vi "UpdateClassApperance.vi"(0 "ClassRefIn":refnum<vi>, 2 "ClassType(Class)":T1, 5 "error in (no error)":errorcluster) -> (14 "ClassRefOut":refnum<vi>, 19 "error out":errorcluster)   [LabVIEW 2020, in "ClassWriter.lvclass"]
uses:
  ClassWriter.lvclass
  ClassApperanceType.ctl
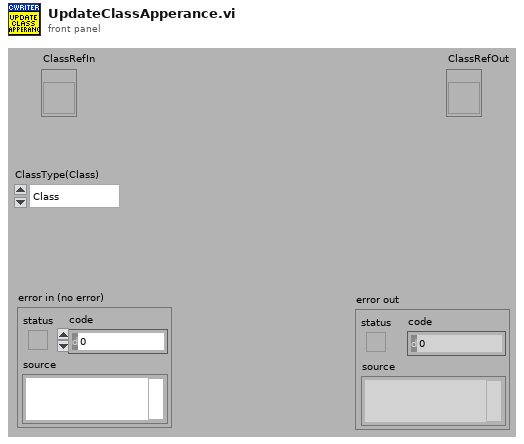
[diagram p1: front panel]
types:
  T1 = typedef "ClassApperanceType.ctl" = enum16{"Class", "AF-MessageClass", "Interface"}
  T2 = typedef "GOOP_WireConfigurationType.ctl" = cluster{"Edge thickness":i32, "Edge color":u32, "Center thickness":i32, "Center pattern":T3, "CenterColor1":u32, "CenterColor2":u32, "Tunnels and terminals colors":u32}
  T3 = typedef "GOOP_WirePattern.ctl" = enum16{"Solid", "Large dash", "Small dash"}
  T4 = typedef "BaseProvider_IniFileSettings.ctl" = cluster{"ClassFolderSuffix":string, "InterfaceFolderSuffix":string, "InterfaceIcon":string, "FileNamingOption":T5, "DynamicDispatchStartValue":bool}
  T5 = typedef "BaseProvider_FileNamingOption.ctl" = enum16{"CamelCase", "Space", "Underscore"}
  T6 = cluster{"Foreground Color":u32, "Background Color":u32, "Fill Pattern":cluster{"Row 0":u8, "Row 1":u8, "Row 2":u8, "Row 3":u8, "Row 4":u8, "Row 5":u8, "Row 6":u8, "Row 7":u8}, "Width":i16, "Mode":enum16{"Copy", "Or", "Exclusive Or", "Bit Clear", "Not Copy", "Not Or", "Nor Exclusive Or", "Not Bit Clear"}, "Style":enum32{"Solid", "Dash", "Dot", "Dash Dot", "Dash Dot Dot"}, "Fill Rule":enum32{"Even Odd", "Winding"}, "End Caps":enum32{"Default", "Flat"}}[]
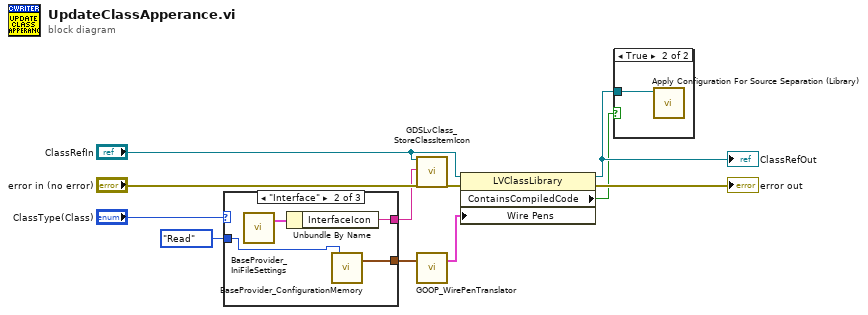
[diagram p0: block diagram]
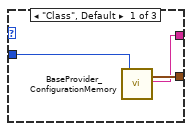
[diagram p3: hidden frame]
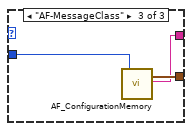
[diagram p4: hidden frame]
diagram:
  n1 = case shown="\"Interface\"" "ClassType(Class)" {
    tunnel: [w14 w18 w20] -> w11
    tunnel: [w13 w15 w19] -> w7
    tunnel: enum16{"Read", "Load", "Save", "Set"}."Read" ("Action") -> [w12 w17 w21]
    frame "Class", Default {
      n2 = call "BaseProvider_ConfigurationMemory.vi"("Action"=w12) -> ("WireConfigurationOut"=w14:T2, "IconOut"=w13:string)  [unwired: 12 in, 5 out]
    }
    frame "Interface" {
      n3 = call "BaseProvider_IniFileSettings.vi"() -> ("IniFileSettings"=w16:T4)  [unwired: 18 in, 1 out]
      n4 = Unbundle By Name(w16) -> ("InterfaceIcon"=w15:string)
      n5 = call "BaseProvider_ConfigurationMemory.vi"("Action"=w17) -> ("WireConfigurationOut"=w18:T2)  [unwired: 12 in, 6 out]
    }
    frame "AF-MessageClass" {
      n6 = call "AF_ConfigurationMemory.vi"("Action"=w21) -> ("AF_MessaageWireConfigurationOut"=w20:T2, "IconOut"=w19:string)  [unwired: 15 in, 2 out]
    }
  }
  n7 = call "GDSLvClass_StoreClassItemIcon.vi"("Library Refnum"="ClassRefIn", "ClassItemIconName"=w7, "error in (no error)"="error in (no error)") -> ("error out"=w9:errorcluster)  [unwired: 15 in, 1 out]
  n8 = call "GOOP_WirePenTranslator.vi"("WireConfigurationIn"=w11) -> ("WirePensOut"=w10:T6)  [unwired: 17 in, 1 out]
  n9 = property class="LVClassLibrary"(reference="ClassRefIn", error in=w9, "Wire Pens"=w10) -> (reference out=w3:refnum<vi>, error out=→"error out":errorcluster, "ContainsCompiledCode"=w1:bool)
  "ClassRefOut" <- w3
  n10 = case shown="True" w1 {
    tunnel: w3 -> [_ w22]
    frame False {
    }
    frame True {
      n11 = call <vilib>:"Apply Configuration For Source Separation (Library).vi"("Library in"=w22) -> ()  [unwired: 9 in, 2 out]
    }
  }
